vi "PWM.vi"(8 "error in (no error)":errorcluster, 10 "power":dbl[](array[numeric])=[0.0, 0.0] format="%#_13g", 11 "Enable":bool[](array[boolean])=[TRUE, TRUE]) -> (0 "error out":errorcluster)   [LabVIEW 2019]
uses:
  <vilib>/myRIO/Instrument Drivers/Onboard IO/PWM/typedefs/PWM Reference.ctl
  <vilib>/myRIO/Common/Instrument Driver Framework/Utilities/typedefs/myRIO Generic Hardware Reference.ctl
  <vilib>/myRIO/Common/Instrument Driver Framework/Utilities/typedefs/Hardware Version Enum.ctl
  <vilib>/myRIO/Common/Instrument Driver Framework/Utilities/typedefs/myRIO v1.0 Reference.ctl
  <vilib>/myRIO/Common/Instrument Driver Framework/Utilities/typedefs/Generic FPGA Reference.ctl
  <vilib>/myRIO/Common/Instrument Driver Framework/myRIO v1.0/PWM/typedefs/PWM Channels Enum.ctl
  <vilib>/myRIO/Instrument Drivers/Onboard IO/PWM/typedefs/PWM Configuration.ctl
  <vilib>/userDefined/High Color/nirio_resource_hc.ctl
  <vilib>/myRIO/Instrument Drivers/Onboard IO/DIO/typedefs/DIO Reference.ctl
  <vilib>/myRIO/Common/Instrument Driver Framework/myRIO v1.0/DIO/typedefs/DIO Channels List.ctl
  <vilib>/myRIO/Common/Instrument Driver Framework/myRIO v1.0/DIO/typedefs/DIO Channels Enum.ctl
  <vilib>/myRIO/Common/Instrument Driver Framework/Utilities/vis/Is FPGA Ref Available.vi
  <vilib>/myRIO/Instrument Drivers/Onboard IO/PWM/vis/Set Duty Cycle and Frequency.vi
  <vilib>/myRIO/Common/Instrument Driver Framework/myRIO v1.0/DIO/vis/myRIO v1.1 Open DIO.vi
  <vilib>/myRIO/Instrument Drivers/Onboard IO/DIO/vis/Write.vi
  <vilib>/myRIO/Common/Instrument Driver Framework/Utilities/vis/Validate Channels.vi
  <vilib>/myRIO/Common/Instrument Driver Framework/myRIO v1.0/DIO/vis/myRIO v1.0 Reserve DIO.vi
  <vilib>/myRIO/Common/Instrument Driver Framework/myRIO v1.0/Resource Manager/vis/myRIO v1.0 Reserve Channel List.vi
  <vilib>/myRIO/Common/Instrument Driver Framework/myRIO v1.0/DIO/vis/myRIO v1.0 Build MUX Configuration DIO.vi
  <vilib>/myRIO/Common/Instrument Driver Framework/myRIO v1.0/Resource Manager/vis/myRIO v1.0 Create Configuration List.vi
  <vilib>/myRIO/Common/Instrument Driver Framework/myRIO v1.0/Resource Manager/vis/myRIO v1.0 Reserve Channel.vi
  <vilib>/myRIO/Common/Instrument Driver Framework/myRIO v1.0/Resource Manager/vis/myRIO v1.0 Unreserve Channel.vi
  <vilib>/myRIO/Common/Instrument Driver Framework/myRIO v1.0/Resource Manager/vis/myRIO v1.0 Build Mutex Name.vi
  <vilib>/Utility/VariantDataType/GetNumericInfo.vi
  <vilib>/Utility/error.llb/Error Cluster From Error Code.vi
  <vilib>/myRIO/Common/Instrument Driver Framework/myRIO v1.0/myRIO v1.1 Open.vi
  <vilib>/myRIO/Common/Instrument Driver Framework/Utilities/vis/IO Manager.vi
  <vilib>/myRIO/Common/Instrument Driver Framework/Utilities/vis/Configuration Manager.vi
  <vilib>/myRIO/Common/Instrument Driver Framework/myRIO v1.0/Resource Manager/vis/myRIO v1.0 Configure IO.vi
  <vilib>/myRIO/Common/Instrument Driver Framework/myRIO v1.0/myRIO v1.0 Close.vi
  <vilib>/myRIO/Common/Instrument Driver Framework/myRIO v1.0/DIO/vis/myRIO v1.0 Write DIO.vi
  <vilib>/myRIO/Express VI/Onboard IO/PWM/PWM Express VI.xnode
  <vilib>/myRIO/Instrument Drivers/Onboard IO/PWM/vis/myRIO PWM Open.xnode
  <vilib>/myRIO/Express VI/Onboard IO/DO/DO Express VI.xnode
  <vilib>/myRIO/Instrument Drivers/Onboard IO/DIO/vis/myRIO DIO Open.xnode
  <vilib>/myRIO/Instrument Drivers/Onboard IO/PWM/PWM.lvlib
  <vilib>/myRIO/Instrument Drivers/Onboard IO/DIO/DIO.lvlib
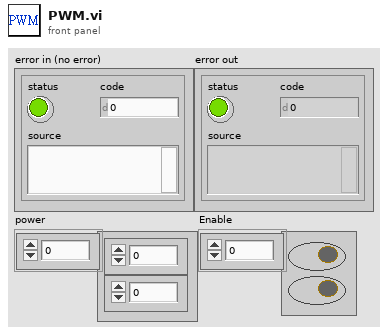
[diagram p1: front panel]
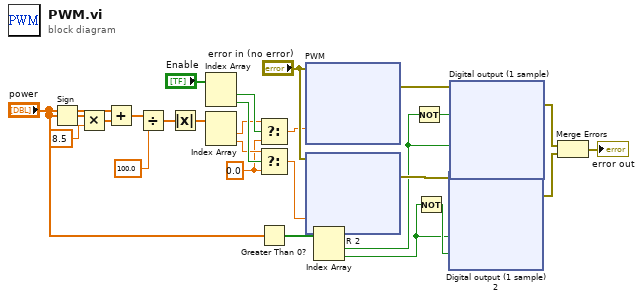
[diagram p0: block diagram]
diagram:
  w8 = 0.0 ("y")
  n1 = Sign(1:"power") -> (0:w26:dbl[])
  n2 = Multiply(x=w26, y=8.5) -> (x*y=w25:dbl[])
  n3 = Add(x="power", y=w25) -> (x+y=w4:dbl[])
  n4 = Divide(x=w4, y=100.0) -> (x/y=w1:dbl[])
  n5 = Absolute Value(x=w1) -> (abs(x)=w2:dbl[])
  n6 = Index Array(array="Enable") -> (element #1=w11:bool, element #2=w12:bool)  [unwired: 2 in]
  n7 = Index Array(array=w2) -> (element #1=w10:dbl, element #2=w9:dbl)  [unwired: 2 in]
  n8 = Select(t=w10, s=w11, f=w8) -> (s? t:f=w7:dbl)
  n9 = Select(t=w9, s=w12, f=w8) -> (s? t:f=w14:dbl)
  n10 = Greater Than 0?(x="power") -> (x > 0?=w21:bool[])
  n11 = xnode "PWM"("Duty Cycle"=w7, "error in (no error)"="error in (no error)") -> ("error out"=w23:errorcluster)
  n12 = xnode "R 2"("Duty Cycle"=w14, "error in (no error)"="error in (no error)") -> ("error out"=w22:errorcluster)
  n13 = Index Array(array=w21) -> (element #1=w15:bool, element #2=w19:bool)  [unwired: 2 in]
  n14 = Not(x=w15) -> (.not. x?=w5:bool)
  n15 = Not(x=w19) -> (.not. x?=w20:bool)
  n16 = xnode "Digital output (1 sample) 2"("INA (A/DIO13 (Pin 26))"=w19, "INB (A/DIO3 (Pin 17))"=w20, "error in (no error)"=w22) -> ("error out"=w17:errorcluster)
  n17 = xnode ("Digital output (1 sample)")("INA (A/DIO2 (Pin 15))"=w15, "INB (A/DIO0 (Pin 11))"=w5, "error in (no error)"=w23) -> ("error out"=w18:errorcluster)
  n18 = Merge Errors(w18, w17) -> (→"error out":errorcluster)
